vi "OFDM_SuperpositionedBitDetectV2.vi"(5 "Alpha":dbl, 8 "error in (no error)":errorcluster, 9 "Modulation type LP":enum16{"QPSK(4QAM)", "64QAM", "16QAM", "BPSK"}(ring), 10 "Modulation type":enum16{"QPSK(4QAM)", "64QAM", "16QAM", "BPSK"}(ring), 11 "Input symbols":cdb[](array[numeric]) format="%.2f") -> (0 "error out":errorcluster, 1 "OutputbitsHP":i8[](array[numeric]) caption="Output bits", 3 "OutputbitsLP":i8[](array[numeric]) caption="Output bits")   [LabVIEW 2022 SP3]
uses:
  <vilib>/addons/Modulation/Digital/General/MT Map QAM Symbols to Bits.vi
  <vilib>/addons/Modulation/Digital/General/MT Map Bits to QAM Symbols.vi
  <vilib>/addons/Modulation/Digital/General/MT Map PSK Symbols to Bits.vi
  <vilib>/addons/Modulation/Digital/General/MT Map Bits to PSK Symbols.vi
  <vilib>/addons/Modulation/niDMT.lvlib
panel:
  out "x-y":cdb[](array[numeric])
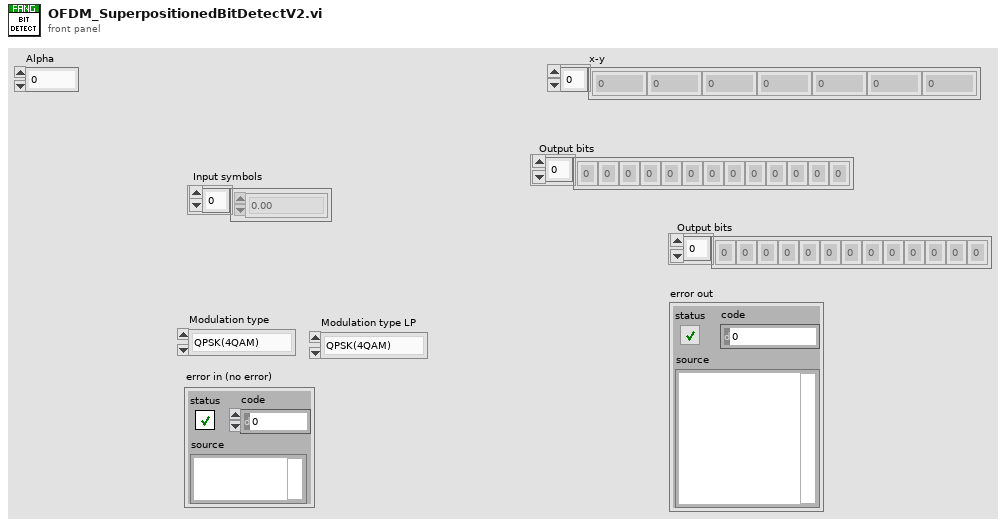
[diagram p1: front panel]
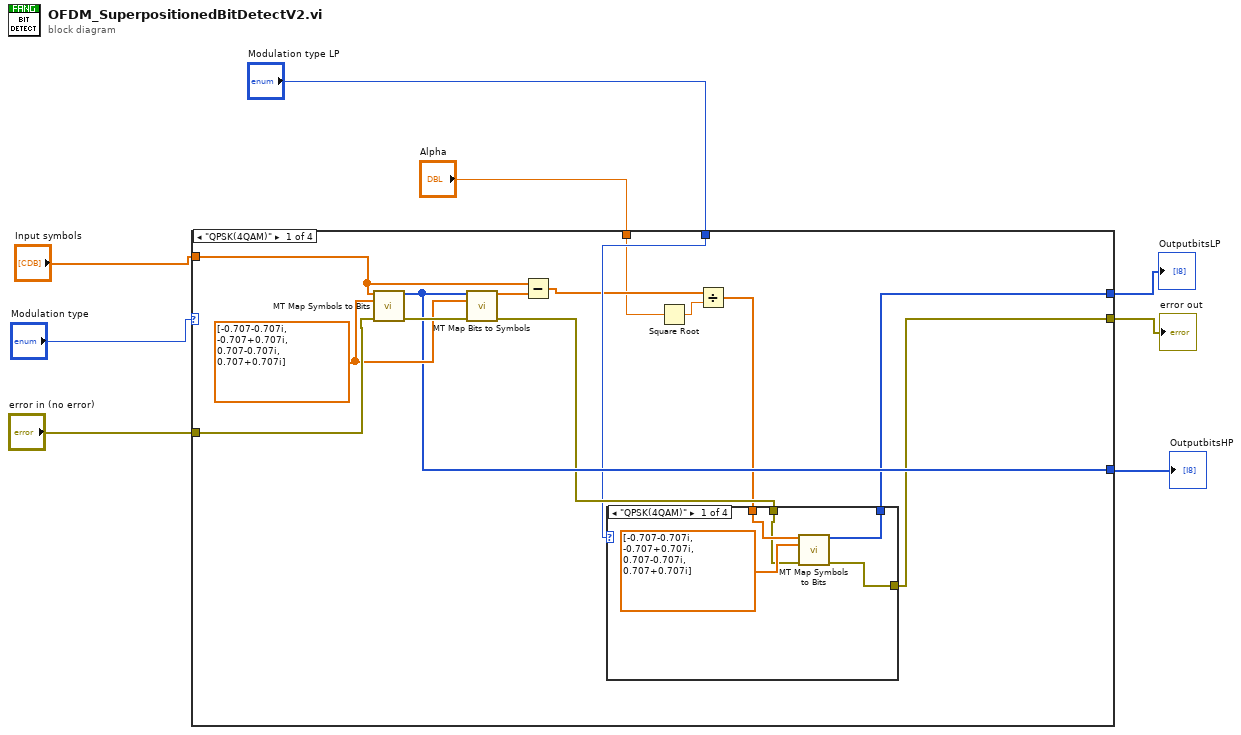
[diagram p0: block diagram]
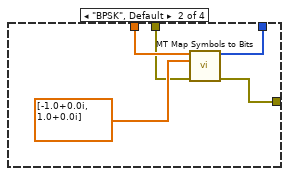
[diagram p2: hidden frame]
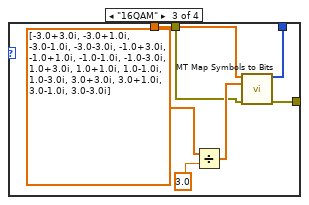
[diagram p3: hidden frame]
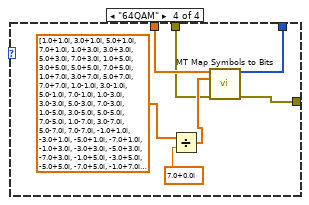
[diagram p4: hidden frame]
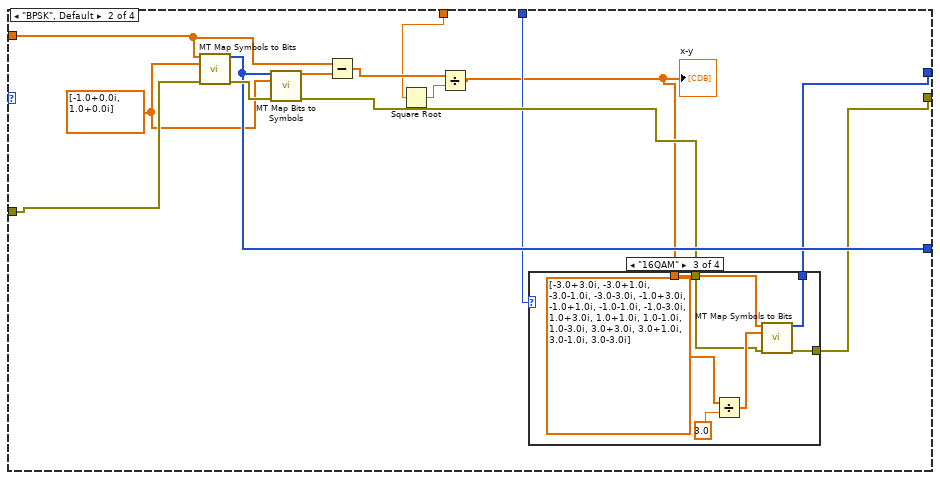
[diagram p5: hidden frame]
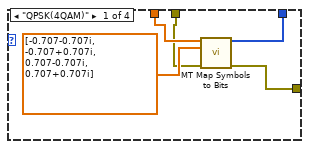
[diagram p6: hidden frame]
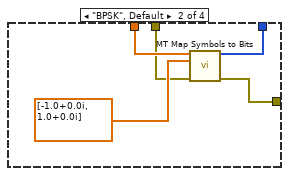
[diagram p7: hidden frame]
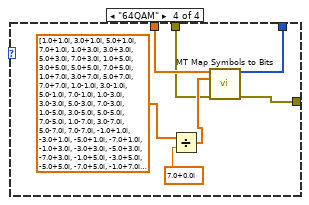
[diagram p8: hidden frame]
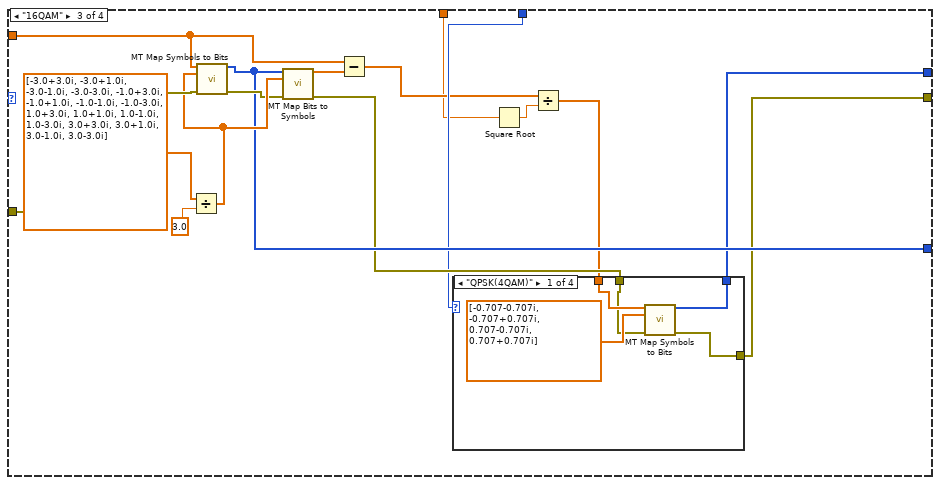
[diagram p9: hidden frame]
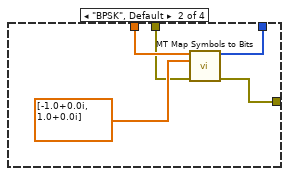
[diagram p10: hidden frame]
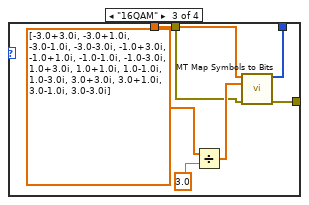
[diagram p11: hidden frame]
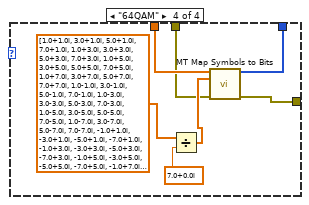
[diagram p12: hidden frame]
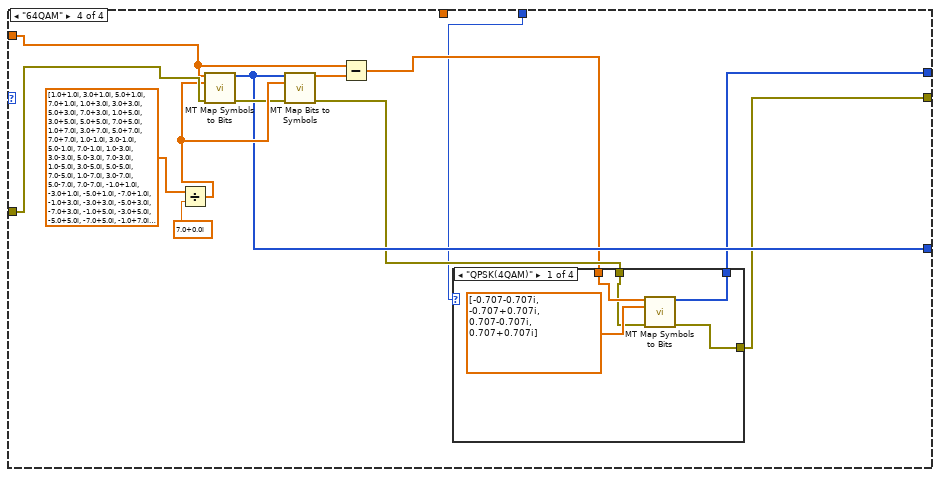
[diagram p13: hidden frame]
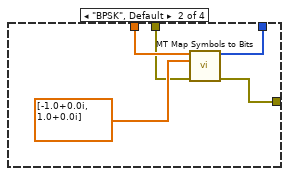
[diagram p14: hidden frame]
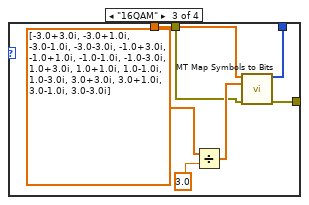
[diagram p15: hidden frame]
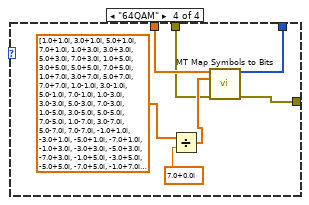
[diagram p16: hidden frame]
diagram:
  n1 = case shown="\"QPSK(4QAM)\"" "Modulation type" {
    tunnel: "Input symbols" -> [w19 w57 w95 w132]
    tunnel: "error in (no error)" -> [w22 w60 w100 w135]
    tunnel: [w14 w54 w90 w127] -> w5
    tunnel: [w15 w53 w91 w128] -> w4
    tunnel: [w17 w56 w93 w130] -> w3
    tunnel: "Modulation type LP" -> [w13 w51 w89 w125]
    tunnel: "Alpha" -> [w9 w47 w85 _]
    frame "QPSK(4QAM)" {
      w18 = cdb[] [-0.707-0.707i, -0.707+0.707i, 0.707-0.707i, 0.707+0.707i] ("symbol map")
      n2 = call-poly <vilib>:"MT Map Symbols to Bits.vi"("symbols"=w19, "symbol map"=w18, "error in (no error)"=w22) -> ("output bit stream"=w17:i8[], "error out"=w21:errorcluster)  [unwired: 11 in]
      n3 = call-poly <vilib>:"MT Map Bits to Symbols.vi"("input bit stream"=w17, "symbol map"=w18, "error in (no error)"=w21) -> ("symbols"=w20:cdb[], "error out"=w16:errorcluster)  [unwired: 11 in]
      n4 = Subtract(x=w19, y=w20) -> (x-y=w10:cdb[])
      n5 = Square Root(x=w9) -> (sqrt(x)=w12:dbl)
      n6 = Divide(x=w10, y=w12) -> (x/y=w11:cdb[])
      n7 = case shown="\"QPSK(4QAM)\"" w13 {
        tunnel: w11 -> [w26 w31 w36 w43]
        tunnel: [w24 w30 w35 w41] -> w14
        tunnel: [w23 w28 w34 w40] -> w15
        tunnel: w16 -> [w25 w29 w33 w42]
        frame "QPSK(4QAM)" {
          n8 = call-poly <vilib>:"MT Map Symbols to Bits.vi"("symbols"=w26, "symbol map"=cdb[] [-0.707-0.707i, -0.707+0.707i, 0.707-0.707i, 0.707+0.707i], "error in (no error)"=w25) -> ("output bit stream"=w24:i8[], "error out"=w23:errorcluster)  [unwired: 11 in]
        }
        frame "BPSK", Default {
          n9 = call-poly <vilib>:"MT Map Symbols to Bits.vi"("symbols"=w31, "symbol map"=cdb[] [-1.0+0.0i, 1.0+0.0i], "error in (no error)"=w29) -> ("output bit stream"=w30:i8[], "error out"=w28:errorcluster)  [unwired: 11 in]
        }
        frame "16QAM" {
          n10 = Divide(x=cdb[] [-3.0+3.0i, -3.0+1.0i, -3.0-1.0i, -3.0-3.0i, -1.0+3.0i, -1.0+1.0i, -1.0-1.0i, -1.0-3.0i, 1.0+3.0i, 1.0+1.0i, 1.0-1.0i, 1.0-3.0i, 3.0+3.0i, 3.0+1.0i, 3.0-1.0i, 3.0-3.0i] ("symbol map"), y=3.0) -> (x/y=w37:cdb[])
          n11 = call-poly <vilib>:"MT Map Symbols to Bits.vi"("symbols"=w36, "symbol map"=w37, "error in (no error)"=w33) -> ("output bit stream"=w35:i8[], "error out"=w34:errorcluster)  [unwired: 11 in]
        }
        frame "64QAM" {
          n12 = Divide(x=cdb[] [1.0+1.0i, 3.0+1.0i, 5.0+1.0i, 7.0+1.0i, 1.0+3.0i, 3.0+3.0i, 5.0+3.0i, 7.0+3.0i, 1.0+5.0i, 3.0+5.0i, 5.0+5.0i, 7.0+5.0i, 1.0+7.0i, 3.0+7.0i, 5.0+7.0i, 7.0+7.0i, 1.0-1.0i, 3.0-1.0i, 5.0-1.0i, 7.0-1.0i, 1.0-3.0i, 3.0-3.0i, 5.0-3.0i, 7.0-3.0i, 1.0-5.0i, 3.0-5.0i, 5.0-5.0i, 7.0-5.0i, 1.0-7.0i, 3.0-7.0i, 5.0-7.0i, 7.0-7.0i, -1.0+1.0i, -3.0+1.0i, -5.0+1.0i, -7.0+1.0i, -1.0+3.0i, -3.0+3.0i, -5.0+3.0i, -7.0+3.0i, -1.0+5.0i, -3.0+5.0i, -5.0+5.0i, -7.0+5.0i, -1.0+7.0i, -3.0+7.0i, -5.0+7.0i, -7.0+7.0i, -1.0-1.0i, -3.0-1.0i, -5.0-1.0i, -7.0-1.0i, -1.0-3.0i, -3.0-3.0i, -5.0-3.0i, -7.0-3.0i, -1.0-5.0i, -3.0-5.0i, -5.0-5.0i, -7.0-5.0i, -1.0-7.0i, -3.0-7.0i, -5.0-7.0i, -7.0-7.0i] ("appended array"), y=cdb 7.0+0.0i) -> (x/y=w44:cdb[])
          n13 = call-poly <vilib>:"MT Map Symbols to Bits.vi"("symbols"=w43, "symbol map"=w44, "error in (no error)"=w42) -> ("output bit stream"=w41:i8[], "error out"=w40:errorcluster)  [unwired: 11 in]
        }
      }
    }
    frame "BPSK", Default {
      w55 = cdb[] [-1.0+0.0i, 1.0+0.0i] ("symbol map")
      n14 = call-poly <vilib>:"MT Map Symbols to Bits.vi"("symbols"=w57, "symbol map"=w55, "error in (no error)"=w60) -> ("output bit stream"=w56:i8[], "error out"=w59:errorcluster)  [unwired: 11 in]
      n15 = call-poly <vilib>:"MT Map Bits to Symbols.vi"("input bit stream"=w56, "symbol map"=w55, "error in (no error)"=w59) -> ("symbols"=w58:cdb[], "error out"=w52:errorcluster)  [unwired: 11 in]
      n16 = Subtract(x=w57, y=w58) -> (x-y=w50:cdb[])
      n17 = Square Root(x=w47) -> (sqrt(x)=w48:dbl)
      n18 = Divide(x=w50, y=w48) -> (x/y=w49:cdb[])
      "x-y" <- w49
      n19 = case shown="\"16QAM\"" w51 {
        tunnel: w49 -> [w64 w69 w74 w81]
        tunnel: [w62 w68 w73 w79] -> w54
        tunnel: [w61 w66 w72 w78] -> w53
        tunnel: w52 -> [w63 w67 w71 w80]
        frame "QPSK(4QAM)" {
          n20 = call-poly <vilib>:"MT Map Symbols to Bits.vi"("symbols"=w64, "symbol map"=cdb[] [-0.707-0.707i, -0.707+0.707i, 0.707-0.707i, 0.707+0.707i], "error in (no error)"=w63) -> ("output bit stream"=w62:i8[], "error out"=w61:errorcluster)  [unwired: 11 in]
        }
        frame "BPSK", Default {
          n21 = call-poly <vilib>:"MT Map Symbols to Bits.vi"("symbols"=w69, "symbol map"=cdb[] [-1.0+0.0i, 1.0+0.0i], "error in (no error)"=w67) -> ("output bit stream"=w68:i8[], "error out"=w66:errorcluster)  [unwired: 11 in]
        }
        frame "16QAM" {
          n22 = Divide(x=cdb[] [-3.0+3.0i, -3.0+1.0i, -3.0-1.0i, -3.0-3.0i, -1.0+3.0i, -1.0+1.0i, -1.0-1.0i, -1.0-3.0i, 1.0+3.0i, 1.0+1.0i, 1.0-1.0i, 1.0-3.0i, 3.0+3.0i, 3.0+1.0i, 3.0-1.0i, 3.0-3.0i] ("symbol map"), y=3.0) -> (x/y=w75:cdb[])
          n23 = call-poly <vilib>:"MT Map Symbols to Bits.vi"("symbols"=w74, "symbol map"=w75, "error in (no error)"=w71) -> ("output bit stream"=w73:i8[], "error out"=w72:errorcluster)  [unwired: 11 in]
        }
        frame "64QAM" {
          n24 = Divide(x=cdb[] [1.0+1.0i, 3.0+1.0i, 5.0+1.0i, 7.0+1.0i, 1.0+3.0i, 3.0+3.0i, 5.0+3.0i, 7.0+3.0i, 1.0+5.0i, 3.0+5.0i, 5.0+5.0i, 7.0+5.0i, 1.0+7.0i, 3.0+7.0i, 5.0+7.0i, 7.0+7.0i, 1.0-1.0i, 3.0-1.0i, 5.0-1.0i, 7.0-1.0i, 1.0-3.0i, 3.0-3.0i, 5.0-3.0i, 7.0-3.0i, 1.0-5.0i, 3.0-5.0i, 5.0-5.0i, 7.0-5.0i, 1.0-7.0i, 3.0-7.0i, 5.0-7.0i, 7.0-7.0i, -1.0+1.0i, -3.0+1.0i, -5.0+1.0i, -7.0+1.0i, -1.0+3.0i, -3.0+3.0i, -5.0+3.0i, -7.0+3.0i, -1.0+5.0i, -3.0+5.0i, -5.0+5.0i, -7.0+5.0i, -1.0+7.0i, -3.0+7.0i, -5.0+7.0i, -7.0+7.0i, -1.0-1.0i, -3.0-1.0i, -5.0-1.0i, -7.0-1.0i, -1.0-3.0i, -3.0-3.0i, -5.0-3.0i, -7.0-3.0i, -1.0-5.0i, -3.0-5.0i, -5.0-5.0i, -7.0-5.0i, -1.0-7.0i, -3.0-7.0i, -5.0-7.0i, -7.0-7.0i] ("appended array"), y=cdb 7.0+0.0i) -> (x/y=w82:cdb[])
          n25 = call-poly <vilib>:"MT Map Symbols to Bits.vi"("symbols"=w81, "symbol map"=w82, "error in (no error)"=w80) -> ("output bit stream"=w79:i8[], "error out"=w78:errorcluster)  [unwired: 11 in]
        }
      }
    }
    frame "16QAM" {
      n26 = Divide(x=cdb[] [-3.0+3.0i, -3.0+1.0i, -3.0-1.0i, -3.0-3.0i, -1.0+3.0i, -1.0+1.0i, -1.0-1.0i, -1.0-3.0i, 1.0+3.0i, 1.0+1.0i, 1.0-1.0i, 1.0-3.0i, 3.0+3.0i, 3.0+1.0i, 3.0-1.0i, 3.0-3.0i] ("symbol map"), y=3.0) -> (x/y=w97:cdb[])
      n27 = call-poly <vilib>:"MT Map Symbols to Bits.vi"("symbols"=w95, "symbol map"=w97, "error in (no error)"=w100) -> ("output bit stream"=w93:i8[], "error out"=w94:errorcluster)  [unwired: 11 in]
      n28 = call-poly <vilib>:"MT Map Bits to Symbols.vi"("input bit stream"=w93, "symbol map"=w97, "error in (no error)"=w94) -> ("symbols"=w96:cdb[], "error out"=w92:errorcluster)  [unwired: 11 in]
      n29 = Subtract(x=w95, y=w96) -> (x-y=w87:cdb[])
      n30 = Square Root(x=w85) -> (sqrt(x)=w88:dbl)
      n31 = Divide(x=w87, y=w88) -> (x/y=w86:cdb[])
      n32 = case shown="\"QPSK(4QAM)\"" w89 {
        tunnel: w86 -> [w104 w109 w114 w121]
        tunnel: [w102 w108 w113 w119] -> w90
        tunnel: [w101 w106 w112 w118] -> w91
        tunnel: w92 -> [w103 w107 w111 w120]
        frame "QPSK(4QAM)" {
          n33 = call-poly <vilib>:"MT Map Symbols to Bits.vi"("symbols"=w104, "symbol map"=cdb[] [-0.707-0.707i, -0.707+0.707i, 0.707-0.707i, 0.707+0.707i], "error in (no error)"=w103) -> ("output bit stream"=w102:i8[], "error out"=w101:errorcluster)  [unwired: 11 in]
        }
        frame "BPSK", Default {
          n34 = call-poly <vilib>:"MT Map Symbols to Bits.vi"("symbols"=w109, "symbol map"=cdb[] [-1.0+0.0i, 1.0+0.0i], "error in (no error)"=w107) -> ("output bit stream"=w108:i8[], "error out"=w106:errorcluster)  [unwired: 11 in]
        }
        frame "16QAM" {
          n35 = Divide(x=cdb[] [-3.0+3.0i, -3.0+1.0i, -3.0-1.0i, -3.0-3.0i, -1.0+3.0i, -1.0+1.0i, -1.0-1.0i, -1.0-3.0i, 1.0+3.0i, 1.0+1.0i, 1.0-1.0i, 1.0-3.0i, 3.0+3.0i, 3.0+1.0i, 3.0-1.0i, 3.0-3.0i] ("symbol map"), y=3.0) -> (x/y=w115:cdb[])
          n36 = call-poly <vilib>:"MT Map Symbols to Bits.vi"("symbols"=w114, "symbol map"=w115, "error in (no error)"=w111) -> ("output bit stream"=w113:i8[], "error out"=w112:errorcluster)  [unwired: 11 in]
        }
        frame "64QAM" {
          n37 = Divide(x=cdb[] [1.0+1.0i, 3.0+1.0i, 5.0+1.0i, 7.0+1.0i, 1.0+3.0i, 3.0+3.0i, 5.0+3.0i, 7.0+3.0i, 1.0+5.0i, 3.0+5.0i, 5.0+5.0i, 7.0+5.0i, 1.0+7.0i, 3.0+7.0i, 5.0+7.0i, 7.0+7.0i, 1.0-1.0i, 3.0-1.0i, 5.0-1.0i, 7.0-1.0i, 1.0-3.0i, 3.0-3.0i, 5.0-3.0i, 7.0-3.0i, 1.0-5.0i, 3.0-5.0i, 5.0-5.0i, 7.0-5.0i, 1.0-7.0i, 3.0-7.0i, 5.0-7.0i, 7.0-7.0i, -1.0+1.0i, -3.0+1.0i, -5.0+1.0i, -7.0+1.0i, -1.0+3.0i, -3.0+3.0i, -5.0+3.0i, -7.0+3.0i, -1.0+5.0i, -3.0+5.0i, -5.0+5.0i, -7.0+5.0i, -1.0+7.0i, -3.0+7.0i, -5.0+7.0i, -7.0+7.0i, -1.0-1.0i, -3.0-1.0i, -5.0-1.0i, -7.0-1.0i, -1.0-3.0i, -3.0-3.0i, -5.0-3.0i, -7.0-3.0i, -1.0-5.0i, -3.0-5.0i, -5.0-5.0i, -7.0-5.0i, -1.0-7.0i, -3.0-7.0i, -5.0-7.0i, -7.0-7.0i] ("appended array"), y=cdb 7.0+0.0i) -> (x/y=w122:cdb[])
          n38 = call-poly <vilib>:"MT Map Symbols to Bits.vi"("symbols"=w121, "symbol map"=w122, "error in (no error)"=w120) -> ("output bit stream"=w119:i8[], "error out"=w118:errorcluster)  [unwired: 11 in]
        }
      }
    }
    frame "64QAM" {
      n39 = Divide(x=cdb[] [1.0+1.0i, 3.0+1.0i, 5.0+1.0i, 7.0+1.0i, 1.0+3.0i, 3.0+3.0i, 5.0+3.0i, 7.0+3.0i, 1.0+5.0i, 3.0+5.0i, 5.0+5.0i, 7.0+5.0i, 1.0+7.0i, 3.0+7.0i, 5.0+7.0i, 7.0+7.0i, 1.0-1.0i, 3.0-1.0i, 5.0-1.0i, 7.0-1.0i, 1.0-3.0i, 3.0-3.0i, 5.0-3.0i, 7.0-3.0i, 1.0-5.0i, 3.0-5.0i, 5.0-5.0i, 7.0-5.0i, 1.0-7.0i, 3.0-7.0i, 5.0-7.0i, 7.0-7.0i, -1.0+1.0i, -3.0+1.0i, -5.0+1.0i, -7.0+1.0i, -1.0+3.0i, -3.0+3.0i, -5.0+3.0i, -7.0+3.0i, -1.0+5.0i, -3.0+5.0i, -5.0+5.0i, -7.0+5.0i, -1.0+7.0i, -3.0+7.0i, -5.0+7.0i, -7.0+7.0i, -1.0-1.0i, -3.0-1.0i, -5.0-1.0i, -7.0-1.0i, -1.0-3.0i, -3.0-3.0i, -5.0-3.0i, -7.0-3.0i, -1.0-5.0i, -3.0-5.0i, -5.0-5.0i, -7.0-5.0i, -1.0-7.0i, -3.0-7.0i, -5.0-7.0i, -7.0-7.0i] ("appended array"), y=cdb 7.0+0.0i) -> (x/y=w134:cdb[])
      n40 = call-poly <vilib>:"MT Map Symbols to Bits.vi"("symbols"=w132, "symbol map"=w134, "error in (no error)"=w135) -> ("output bit stream"=w130:i8[], "error out"=w131:errorcluster)  [unwired: 11 in]
      n41 = call-poly <vilib>:"MT Map Bits to Symbols.vi"("input bit stream"=w130, "symbol map"=w134, "error in (no error)"=w131) -> ("symbols"=w133:cdb[], "error out"=w129:errorcluster)  [unwired: 11 in]
      n42 = Subtract(x=w132, y=w133) -> (x-y=w126:cdb[])
      n43 = case shown="\"QPSK(4QAM)\"" w125 {
        tunnel: w126 -> [w141 w146 w151 w158]
        tunnel: [w139 w145 w150 w156] -> w127
        tunnel: [w138 w143 w149 w155] -> w128
        tunnel: w129 -> [w140 w144 w148 w157]
        frame "QPSK(4QAM)" {
          n44 = call-poly <vilib>:"MT Map Symbols to Bits.vi"("symbols"=w141, "symbol map"=cdb[] [-0.707-0.707i, -0.707+0.707i, 0.707-0.707i, 0.707+0.707i], "error in (no error)"=w140) -> ("output bit stream"=w139:i8[], "error out"=w138:errorcluster)  [unwired: 11 in]
        }
        frame "BPSK", Default {
          n45 = call-poly <vilib>:"MT Map Symbols to Bits.vi"("symbols"=w146, "symbol map"=cdb[] [-1.0+0.0i, 1.0+0.0i], "error in (no error)"=w144) -> ("output bit stream"=w145:i8[], "error out"=w143:errorcluster)  [unwired: 11 in]
        }
        frame "16QAM" {
          n46 = Divide(x=cdb[] [-3.0+3.0i, -3.0+1.0i, -3.0-1.0i, -3.0-3.0i, -1.0+3.0i, -1.0+1.0i, -1.0-1.0i, -1.0-3.0i, 1.0+3.0i, 1.0+1.0i, 1.0-1.0i, 1.0-3.0i, 3.0+3.0i, 3.0+1.0i, 3.0-1.0i, 3.0-3.0i] ("symbol map"), y=3.0) -> (x/y=w152:cdb[])
          n47 = call-poly <vilib>:"MT Map Symbols to Bits.vi"("symbols"=w151, "symbol map"=w152, "error in (no error)"=w148) -> ("output bit stream"=w150:i8[], "error out"=w149:errorcluster)  [unwired: 11 in]
        }
        frame "64QAM" {
          n48 = Divide(x=cdb[] [1.0+1.0i, 3.0+1.0i, 5.0+1.0i, 7.0+1.0i, 1.0+3.0i, 3.0+3.0i, 5.0+3.0i, 7.0+3.0i, 1.0+5.0i, 3.0+5.0i, 5.0+5.0i, 7.0+5.0i, 1.0+7.0i, 3.0+7.0i, 5.0+7.0i, 7.0+7.0i, 1.0-1.0i, 3.0-1.0i, 5.0-1.0i, 7.0-1.0i, 1.0-3.0i, 3.0-3.0i, 5.0-3.0i, 7.0-3.0i, 1.0-5.0i, 3.0-5.0i, 5.0-5.0i, 7.0-5.0i, 1.0-7.0i, 3.0-7.0i, 5.0-7.0i, 7.0-7.0i, -1.0+1.0i, -3.0+1.0i, -5.0+1.0i, -7.0+1.0i, -1.0+3.0i, -3.0+3.0i, -5.0+3.0i, -7.0+3.0i, -1.0+5.0i, -3.0+5.0i, -5.0+5.0i, -7.0+5.0i, -1.0+7.0i, -3.0+7.0i, -5.0+7.0i, -7.0+7.0i, -1.0-1.0i, -3.0-1.0i, -5.0-1.0i, -7.0-1.0i, -1.0-3.0i, -3.0-3.0i, -5.0-3.0i, -7.0-3.0i, -1.0-5.0i, -3.0-5.0i, -5.0-5.0i, -7.0-5.0i, -1.0-7.0i, -3.0-7.0i, -5.0-7.0i, -7.0-7.0i] ("appended array"), y=cdb 7.0+0.0i) -> (x/y=w159:cdb[])
          n49 = call-poly <vilib>:"MT Map Symbols to Bits.vi"("symbols"=w158, "symbol map"=w159, "error in (no error)"=w157) -> ("output bit stream"=w156:i8[], "error out"=w155:errorcluster)  [unwired: 11 in]
        }
      }
    }
  }
  "OutputbitsLP" <- w5
  "error out" <- w4
  "OutputbitsHP" <- w3
